vi "Write I64.vi"(8 "error in (no error)":errorcluster, 9 "Timeout (ms)":i32, 10 "Data":i64, 11 "CIFTag in":refnum<class "CIF_Iceoryx_Chn_I64.lvclass">) -> (0 "error out":errorcluster, 1 "timed out?":bool, 3 "CIFTag out":refnum<class "CIF_Iceoryx_Chn_I64.lvclass">)   [LabVIEW 2021, in "CIF_Iceoryx_Chn_I64.lvclass"]
uses:
  CIF_Iceoryx_Chn_I64.lvclass
  D:/dev/Packages/CIF_Channels_Core/src/CIFChannels/CIFChannels.lvclass
  D:/dev/Packages/CIF_Channels_Core/src/Iceorxy_Channels/CIF_Iceoryx_BB/CIF_Iceoryx_BB.lvclass
  CIFChannels/CIFChannels.lvclass/CIFChannels.ctl
  CIF_Iceoryx_BB/CIF_Iceoryx_BB.lvclass/CIF_Iceoryx_BB.ctl
  CIF_Iceoryx_Chn_I64.lvclass/CIF_Iceoryx_Chn_I64.ctl
  CIF_Iceoryx_BB/Accessors/Read Writer Reference.vi
  Write I64 Direct.vi/ed0394a0-663f-427f-8194-a1e85751af09.vi
  CIFChannels/Accessors/Read Tag Forced.vi
  <vilib>/CIF Foundation/CIF Iceoryx/SubVIs/Get Path.vi
  <vilib>/CIF Foundation/CIF Iceoryx/SubVIs/Convert Error.vi
  <vilib>/CIF Foundation/CIF Iceoryx/Refnum/BB Writer from Refnum.vi
  <vilib>/CIF Foundation/CIF Iceoryx/SubVIs/Convert Error Core.vi
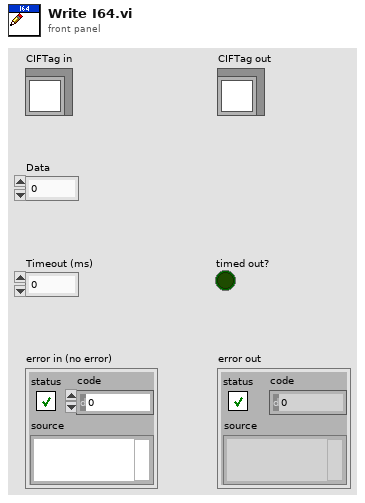
[diagram p1: front panel]
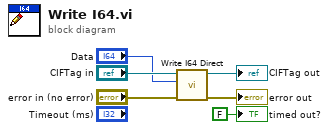
[diagram p0: block diagram]
diagram:
  n1 = call "Write I64 Direct.vi"("error in (no error)"="error in (no error)", "Data"="Data", "CIFTag in"="CIFTag in") -> ("error out"=→"error out":errorcluster, "CIFTag out"=→"CIFTag out":refnum<class "CIF_Iceoryx_Chn_I64.lvclass">)  [unwired: 7 in]
  "timed out?" <- FALSE ("timed out?")
